vi "Create DAQmx Task.vi"(8 "error in (no error)":errorcluster, 11 "DAQmxDI in":refnum<class "DAQmxDI.lvclass">) -> (0 "error out":errorcluster, 3 "DAQmxDI out":refnum<class "DAQmxDI.lvclass">)   [LabVIEW 2020, in "VolatusDAQ.lvlib" / "DAQmxDI.lvclass"]
uses:
  DAQmxDI.lvclass
  C:/dev/lv20CE/relink/lv-volatus/Volatus/Module/Module.lvclass
  lv-vecto/Vecto/Group DBL/Group DBL.lvclass
  C:/dev/lv20CE/relink/lv-vecto/Vecto/Group/Group.lvclass
  Volatus/Module/Module.lvclass/Module.ctl
  DAQmxDI.lvclass/DAQmxDI.ctl
  VolatusConfig/VolatusConfigElement/VolatusConfigElement.lvclass/VolatusConfigElement.ctl
  Volatus/Module/Config.vi
  VolatusConfig/VolatusConfigElement/Element.vi
  VolatusConfig/Group/Group Config.lvclass
  C:/dev/lv20CE/relink/lv-volatus/VolatusConfig/VolatusConfigElement/VolatusConfigElement.lvclass
  VolatusConfig/Task/Task Config.lvclass
  <vilib>/DAQmx/configure/timing.llb/DAQmx Timing (Sample Clock).vi
  <vilib>/DAQmx/create/channels.llb/DAQmx Create Channel (DI-Digital Input).vi
  Volatus/Module/Module.lvclass
  VolatusConfig/VolatusConfigElement/VolatusConfigElement.lvclass
  VolatusDAQConfig/VolatusDAQConfig.lvlib
  C:/dev/lv20CE/relink/lv-volatus/VolatusDAQ/DAQmxDI/DAQmxDI.lvclass
  VolatusDAQ.lvlib
  <resource>/objmgr/daqmx.rc
  C:/dev/lv20CE/relink/lv-volatus/VolatusConfig/Group/Group Config.lvclass
  C:/dev/lv20CE/relink/lv-vecto/Vecto/Group DBL/Group DBL.lvclass
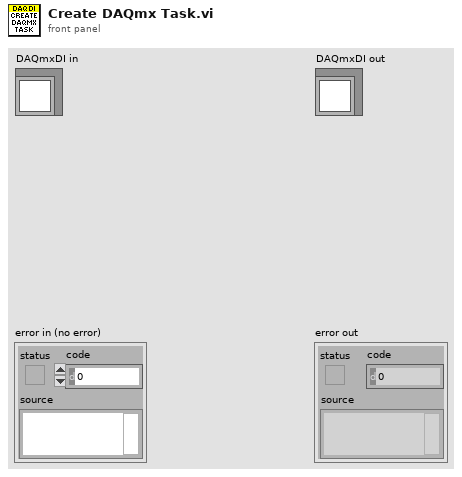
[diagram p1: front panel]
types:
  T1 = typedef "VolatusDAQ.lvlib/DAQmxDI.lvclass/Port Info.ctl" = cluster{"Module Alias":string, "Number":i32, "# Lines":i32, "Lines":map{i32, string}, "Channel Indices":i32[]}
  T2 = typedef "VolatusDAQConfig.lvlib/Sampling Config.ctl" = cluster{"Rate":dbl, "Chunk Size":i32}
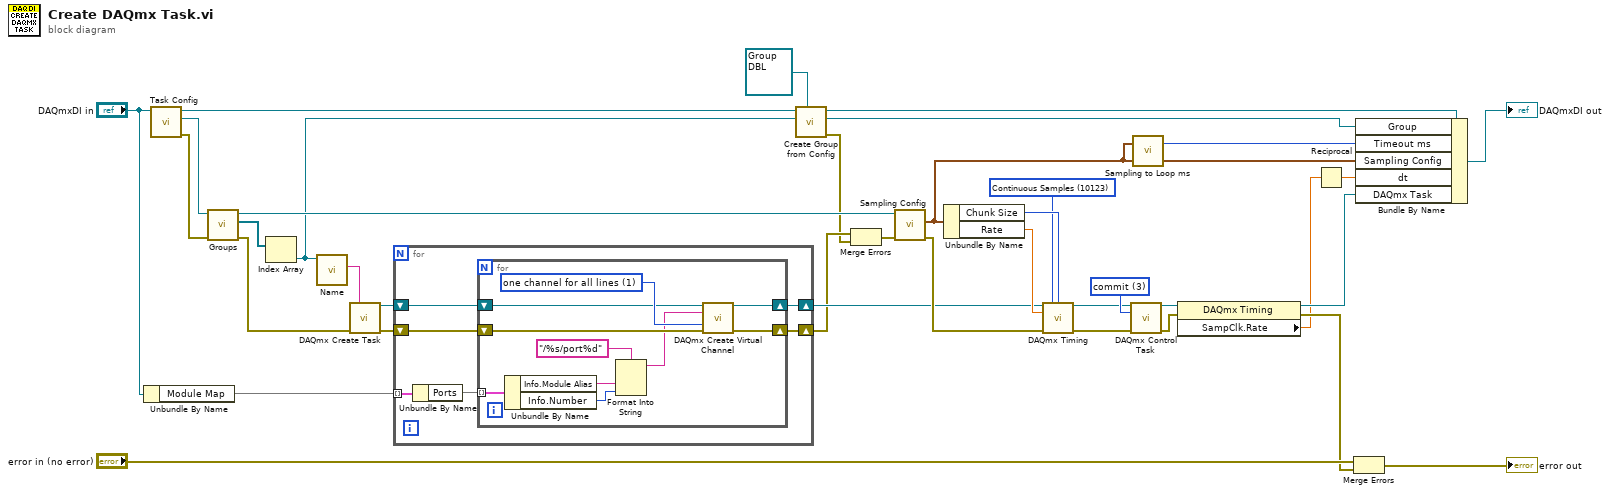
[diagram p0: block diagram]
diagram:
  w20 = 3 items=["verify"=2, "reserve"=4, "commit"=3, "unreserve"=5, "abort"=6] ("action")
  w22 = 10123 items=["Finite Samples"=10178, "Continuous Samples"=10123, "Hardware Timed Single Point"=12522] ("sample mode")
  n1 = Unbundle By Name("DAQmxDI in") -> ("Module Map"=w27:map{string, map{i32, T1}})
  n2 = call "Task Config.vi"("Module in"="DAQmxDI in") -> ("error out"=w35:errorcluster, "Task Config"=w34:refnum<class "Task Config.lvclass">, "Module out"=w31:refnum<class "DAQmxDI.lvclass">)  [unwired: 8 in]
  n3 = call "Groups.vi"("error in (no error)"=w35, "Task in"=w34) -> ("error out"=w37:errorcluster, "Groups"=w33:refnum<class "Group Config.lvclass">[], "Task out"=w23:refnum<class "Task Config.lvclass">)  [unwired: 7 in]
  n4 = Index Array(array=w33) -> (element=w14:refnum<class "Group Config.lvclass">)  [unwired: 1 in]
  n5 = call "Name.vi"("VolatusConfigElement in"=w14) -> ("Name"=w30:string)  [unwired: 8 in, 2 out]
  n6 = call <vilib>:"DAQmx Create Task.vi"("new task name"=w30, "error in"=w37) -> ("task out"=w29:refnum<k21>, "error out"=w28:errorcluster)  [unwired: 12 in]
  n7 = for {
    shift-right: [w39] -> w21
    shift-left: w29 -> [w40]
    shift-right: [w38] -> w11
    shift-left: w28 -> [w41]
    tunnel: w27 -> [w43] mode=indexing
    n8 = Unbundle By Name(w43) -> ("Ports"=w42:map{i32, T1})
    n9 = for {
      tunnel: w42 -> [w53] mode=indexing
      shift-right: [w45] -> w38
      shift-left: w41 -> [w47]
      shift-right: [w44] -> w39
      shift-left: w40 -> [w48]
      w49 = 1 items=["one channel for each line", "one channel for all lines"] ("line grouping")
      n10 = Unbundle By Name(w53) -> ("Info.Module Alias"=w51:string, "Info.Number"=w50:i32)
      n11 = Format Into String(format string="/%s/port%d", w51, w50) -> (resulting string=w46:string)  [unwired: 2 in, 1 out]
      n12 = call-poly <vilib>:"DAQmx Create Virtual Channel.vi"("task in"=w48, "lines"=w46, "line grouping"=w49, "error in"=w47) -> ("task out"=w44:refnum<k21>, "error out"=w45:errorcluster)  [unwired: 10 in]
    }
  }
  n13 = call "Create Group from Config.vi"("Group Type (Abstract)"=refnum<class "Group DBL.lvclass"> refnum ("Vecto.lvlib:Group DBL.lvclass"), "Group Config"=w14, "Module in"=w31) -> ("error out"=w9:errorcluster, "Group"=w12:refnum<class "Group DBL.lvclass">, "Module out"=w15:refnum<class "DAQmxDI.lvclass">)  [unwired: 6 in]
  n14 = Merge Errors(w11, w9) -> (w10:errorcluster)
  n15 = call "Sampling Config.vi"("error in (no error)"=w10, "Task In"=w23) -> ("error out"=w26:errorcluster, "Sampling Config"=w7:T2)  [unwired: 7 in, 1 out]
  n16 = Unbundle By Name(w7) -> ("Chunk Size"=w24:i32, "Rate"=w25:dbl)
  n17 = call-poly <vilib>:"DAQmx Timing.vi"("task/channels in"=w21, "sample mode"=w22, "samples per channel"=w24, "rate"=w25, "error in"=w26) -> ("task out"=w19:refnum<k21>, "error out"=w18:errorcluster)  [unwired: 9 in]
  n18 = call <vilib>:"DAQmx Control Task.vi"("task/channels in"=w19, "action"=w20, "error in"=w18) -> ("task out"=w6:refnum<k21>, "error out"=w5:errorcluster)  [unwired: 11 in]
  n19 = call "Sampling to Loop ms.vi"("Sampling Config"=w7) -> ("Loop Timeout ms"=w8:i32)  [unwired: 6 in]
  n20 = property class="DAQmx Timing"(reference=w6, error in=w5) -> (reference out=w4:refnum<k21>, error out=w3:errorcluster, "SampClk.Rate"=w2:dbl)
  n21 = Reciprocal(x=w2) -> (1/x=w1:dbl)
  n22 = Merge Errors("error in (no error)", w3) -> (→"error out":errorcluster)
  n23 = Bundle By Name(cluster=w15, "Group"=w12, "Timeout ms"=w8, "Sampling Config"=w7, "dt"=w1, "DAQmx Task"=w4) -> (→"DAQmxDI out":refnum<class "DAQmxDI.lvclass">)
